vi "Remove_Disabled_Structure.vi"(8 "error in":errorcluster, 11 "Top Level/Always Included VIs":path[](array[path])) -> (0 "error out":errorcluster)   [LabVIEW 2027, in "Build VIs.lvlib"]
uses:
  <vilib>/Utility/traverseref.llb/TRef TravTarget.ctl
  Build VIs.lvlib
  <vilib>/Utility/traverseref.llb/VI Scripting - Traverse.lvlib
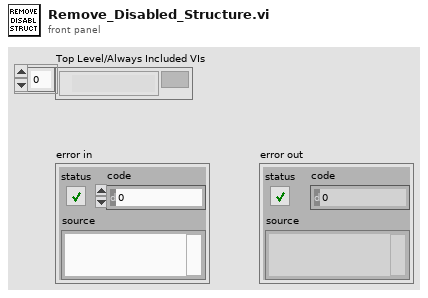
[diagram p1: front panel]
types:
  T1 = typedef "TRef TravTarget.ctl" = enum16{"FP", "BD", "Other"}
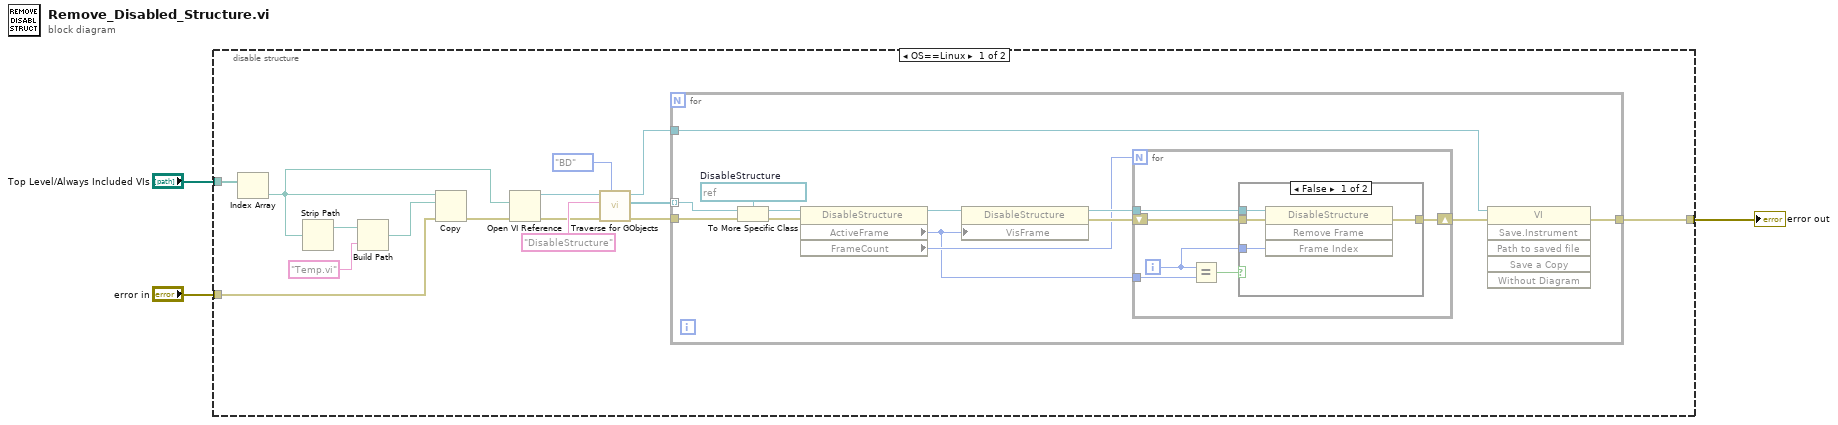
[diagram p0: block diagram]
diagram:
  n1 = disable-structure shown="OS==Linux" {
    disable-tunnel: [w17 w43] -> w3
    disable-tunnel: "Top Level/Always Included VIs" -> [w5 _]
    disable-tunnel: "error in" -> [w4 w43]
    frame condition #0 {
      n2 = Index Array(array=w5) -> (element=w18:path)  [unwired: 1 in]
      n3 = Strip Path(path=w18) -> (stripped path=w13:path)  [unwired: 1 out]
      n4 = Build Path(base path=w13, name or relative path="Temp.vi" ("Class Name")) -> (appended path=w15:path)
      n5 = Copy(8:w4, 10:w15, 11:w18) -> (0:w16:errorcluster)  [unwired: 2 in, 2 out]
      n6 = Open VI Reference(vi path=w18, error in (no error)=w16) -> (vi reference=w6:refnum<vi>, error out=w7:errorcluster)  [unwired: 4 in]
      n7 = call <vilib>:"Traverse for GObjects.vi"("Traverse Target"=TRef_TravTarget."BD", "error in (no error)"=w7, "Class Name"="DisableStructure", "VI Refnum"=w6) -> ("error out"=w10:errorcluster, "References"=w12:refnum<vi>[], "dup VI Refnum"=w11:refnum<vi>)  [unwired: 4 in, 1 out]
      n8 = for {
        tunnel: w10 -> [w29]
        tunnel: [w23] -> w17
        tunnel: w11 -> [w22]
        tunnel: w12 -> [w21] mode=indexing
        w30 = refnum<vi> refnum  # DisableStructure
        n9 = To More Specific Class(target class=w30, reference=w21, error in=w29) -> (specific class reference=w31:refnum<vi>, error out=w28:errorcluster)
        n10 = property class="DisableStructure"(reference=w31, error in=w28) -> (reference out=w27:refnum<vi>, "ActiveFrame"=w19:i16, "FrameCount"=w20:i32)  [unwired: 1 out]
        n11 = property class="DisableStructure"(reference=w27, "VisFrame"=w19) -> (reference out=w26:refnum<vi>, error out=w25:errorcluster)  [unwired: 1 in]
        n12 = for {
          N: w20 -> [_]
          tunnel: w26 -> [w37]
          shift-right: [w35] -> w24
          shift-left: w25 -> [w36]
          tunnel: w19 -> [w34]
          i -> [w33]
          n13 = Equal?(x=w33, y=w34) -> (x = y?=w32:bool)
          n14 = case shown="False" w32 {
            tunnel: w37 -> [w41 _]
            tunnel: w36 -> [w40 w42]
            tunnel: [w39 w42] -> w35
            tunnel: w33 -> [w38 _]
            frame False {
              n15 = invoke class="DisableStructure" method="Remove Frame"(reference=w41, error in=w40, "Frame Index"=w38) -> (error out=w39:errorcluster)  [unwired: 1 in, 3 out]
            }
            frame True {
            }
          }
        }
        n16 = invoke class="VI" method="Save.Instrument"(reference=w22, error in=w24) -> (error out=w23:errorcluster)  [unwired: 4 in, 5 out]
      }
    }
    frame condition #1 (active) {
    }
  }
  "error out" <- w3
